vi "Write (recursive).vi"(7 "LoopData in":T3, 9 "Options":T1, 10 "Anything":variant, 11 "TagPath":string[](array[string])) -> (0 "error out":errorcluster, 3 "Tree Items":T4[](array[typedef]), 5 "LoopData out":T3)   [LabVIEW 2020, in "BlueVariantView.lvlib"]
uses:
  BlueVariantView.lvlib
  API/Typedefs/TreeData.ctl
  LoopData.ctl
  API/Typedefs/Options.ctl
  IsErrorCluster.vi
  SymbolEnumToIndex.vi
  StringArrayToScalar.vi
  <vilib>/Utility/Data Type/Get Cluster Information.vi
  <userlib>/_OpenG.lib/lvdata/lvdata.llb/Array Size(s)__ogtk.vi
  <vilib>/Utility/error.llb/Trim Whitespace.vi
  <vilib>/Utility/error.llb/Error Cluster From Error Code.vi
  <vilib>/Utility/LVClass/Get LV Class Name.vi
  <vilib>/PNR/LabVIEW Composition/Composition/Decompose LabVIEW Object.vi
  <vilib>/PNR/LabVIEW Composition/Composition/Decompose Map.vi
  <vilib>/Utility/Data Type/Get Numeric Information.vi
  <userlib>/_OpenG.lib/lvdata/lvdata.llb/Get Physical Units__ogtk.vi
  <vilib>/ErrorRing/Error Ring.xnode
  <vilib>/Utility/Data Type/NI_Data Type.lvlib
  <vilib>/PNR/LabVIEW Composition/Composition/Composition.lvlib
  API/Typedefs/ValueOptions.ctl
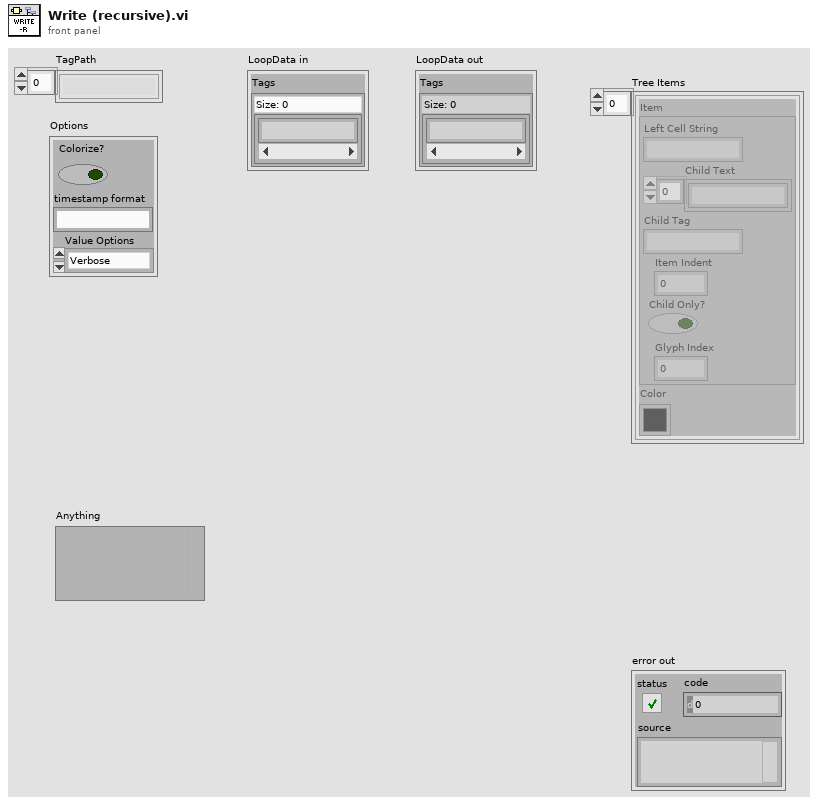
[diagram p1: front panel]
types:
  T1 = typedef "BlueVariantView.lvlib/Options.ctl" = cluster{"Colorize?":bool, "timestamp format":string, "Value Options":T2}
  T2 = typedef "BlueVariantView.lvlib/ValueOptions.ctl" = enum16{"Verbose", "Data only"}
  T3 = typedef "BlueVariantView.lvlib/LoopData.ctl" = cluster{"Tags":set{string}}
  T4 = typedef "BlueVariantView.lvlib/TreeData.ctl" = cluster{"Item":cluster{"Left Cell String":string, "Child Text":string[], "Child Tag":string, "Item Indent":i32, "Child Only?":bool, "Glyph Index":i32}, "Color":u32}
  T5 = typedef "NI_Data Type.lvlib/Data Type.ctl" = enum8{"Invalid Type", "Void", "I8", "I16", "I32", "I64", "U8", "U16", "U32", "U64", "Single Float", "Double Float", "Extended Float", "Single Complex", "Double Complex", "Extended Complex", "Enum U8", "Enum U16", "Enum U32", "Enum U64", "Single Float With Unit", "Double Float With Unit", "Extended Float With Unit", "Single Complex with Unit", "Double Complex with Unit", "Extended Complex with Unit", "Boolean", "String", "Path", "Picture", "Tag", "Array", "Cluster", "Variant", "LV Variant", "Waveform", "Timestamp", "Digital Waveform", "Digital Data", "ExpressData", "Refnum", "External Data", "VI", "Poly VI", "LabVIEW Class Instance", "Fixed Point", "Set Collection", "Map Collection"}
  T6 = typedef "BlueVariantView.lvlib/DecomposedObject.ctl" = cluster{"class name":string, "class version":string, "Private Data":variant}
  T7 = typedef "BlueVariantView.lvlib/DecomposedMap.ctl" = cluster{"Key":variant, "Value":variant}
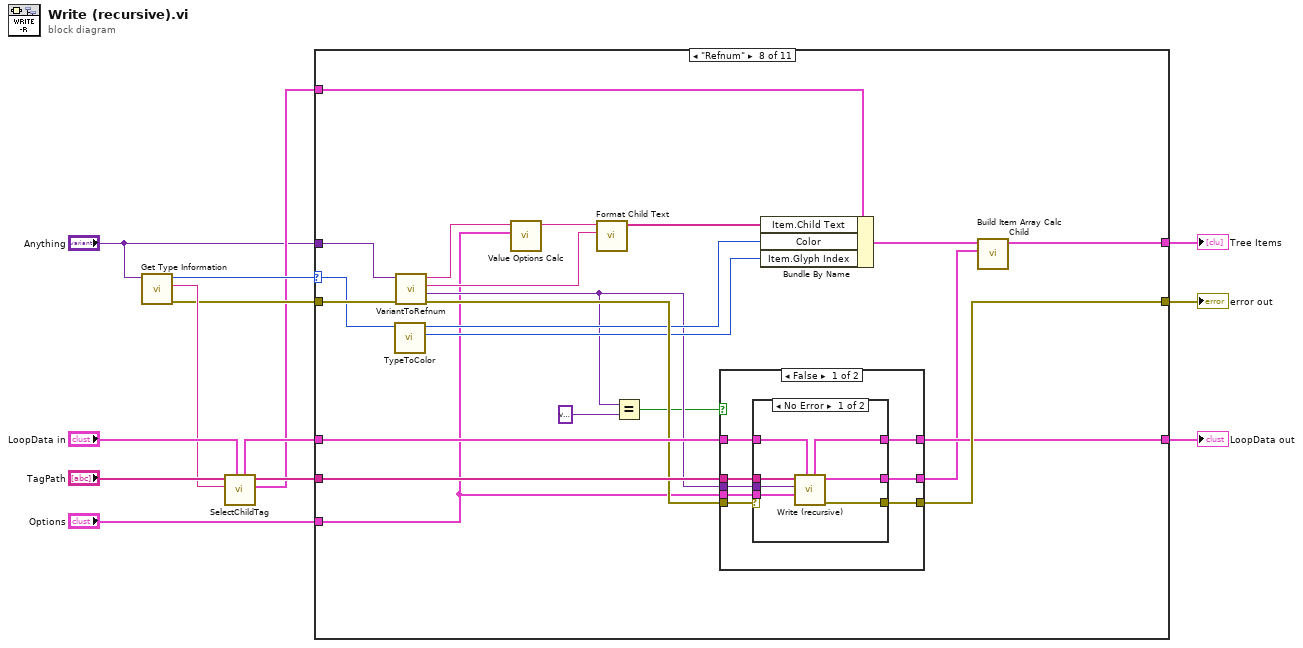
[diagram p0: block diagram]
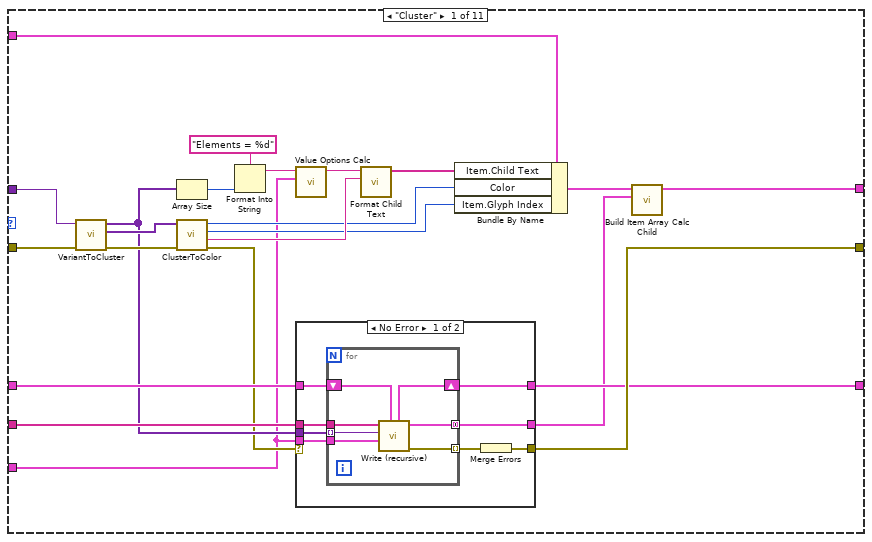
[diagram p2: hidden frame]
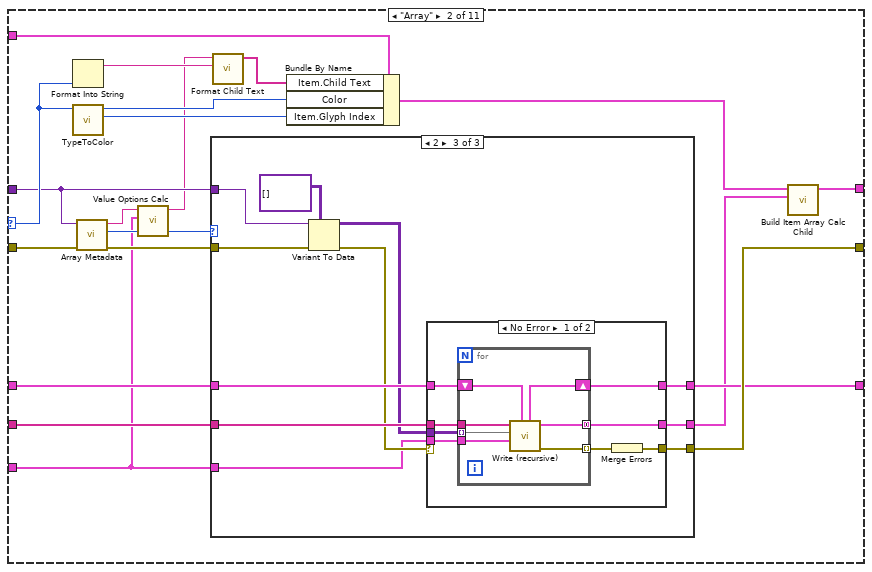
[diagram p4: hidden frame]
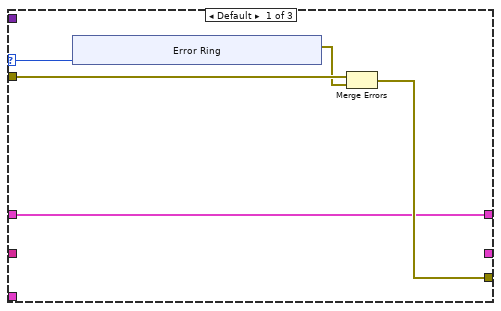
[diagram p5: hidden frame]
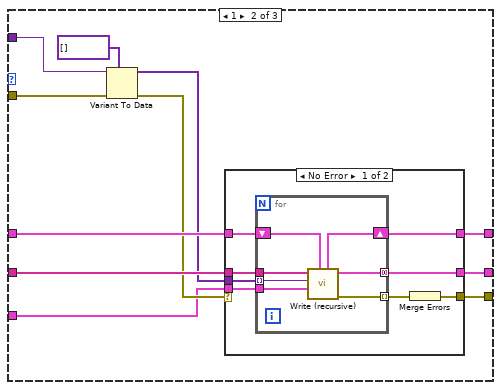
[diagram p6: hidden frame]
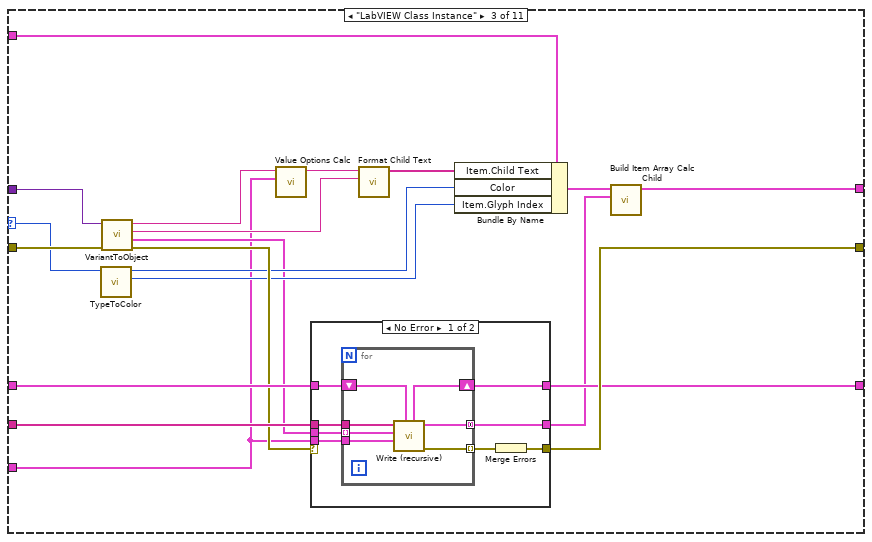
[diagram p9: hidden frame]
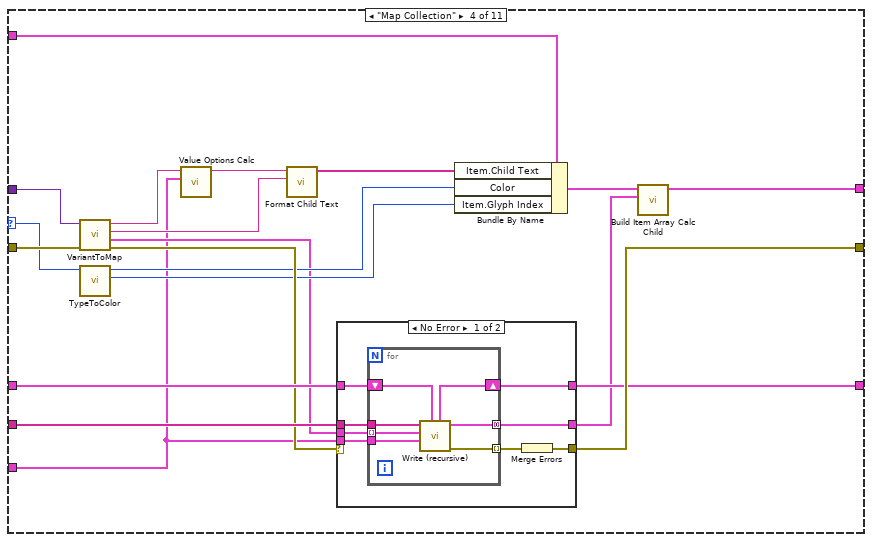
[diagram p11: hidden frame]
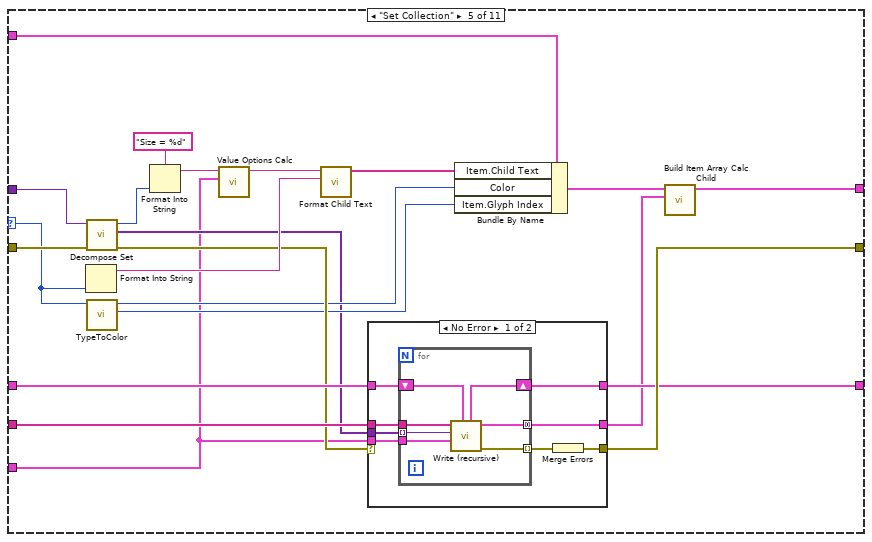
[diagram p13: hidden frame]
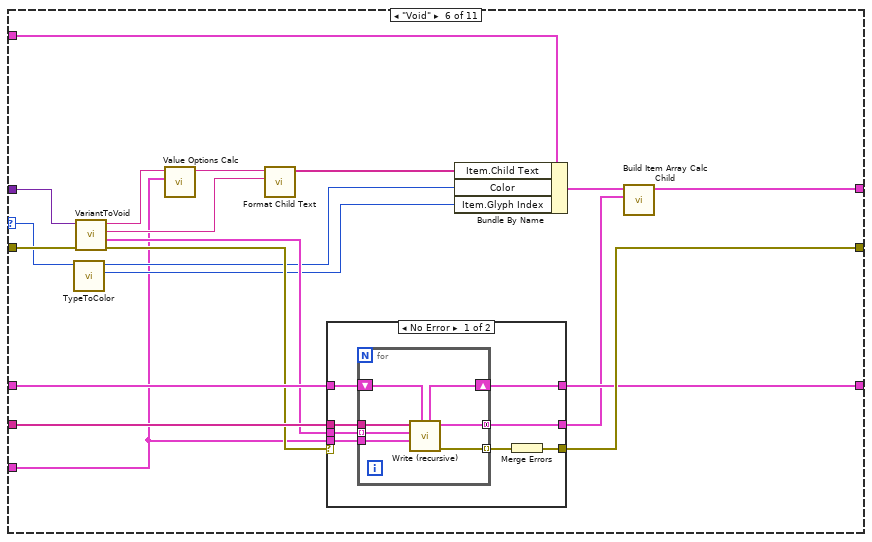
[diagram p15: hidden frame]
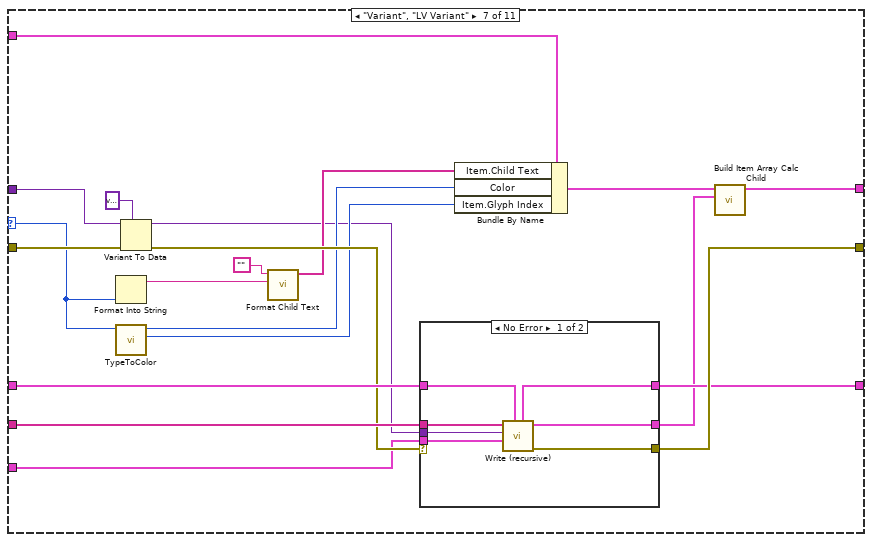
[diagram p17: hidden frame]
diagram:
  n1 = call <vilib>:"Get Type Information.vi"("variant"="Anything") -> ("error out"=w9:errorcluster, "name"=w11:string, "type"=w10:T5)  [unwired: 6 in, 2 out]
  n2 = call "SelectChildTag.vi"("LoopData in"="LoopData in", "Name"=w11, "TagPath in"="TagPath") -> ("Item"=w6:T4, "TagPath out"=w8:string[], "LoopData out"=w7:T3)  [unwired: 6 in]
  n3 = case shown="\"Refnum\"" w10 {
    selector: w10 -> [_ w67 w154 w188 w227 w263 w301 w332 w368 w381 w396]
    tunnel: w9 -> [w36 w68 w156 w193 w229 w269 w305 w337 w371 w383 w399]
    tunnel: w8 -> [w33 w72 w160 w197 w236 w273 w310 w341 _ _ _]
    tunnel: w7 -> [w32 w71 w159 w196 w235 w272 w309 w340 w365 w388 w404]
    tunnel: w6 -> [w23 w69 w157 w194 w233 w270 w307 w338 w374 w392 w408]
    tunnel: "Anything" -> [w35 w65 w155 w192 w228 w268 w306 w336 w370 w385 w398]
    tunnel: [w34 w73 w161 w198 w237 w274 w311 w342 w364 w382 w400] -> w4
    tunnel: [w31 w70 w158 w195 w234 w271 w308 w339 w365 w388 w404] -> w3
    tunnel: [w17 w59 w145 w182 w219 w258 w293 w324 w362 w386 w402] -> w2
    tunnel: "Options" -> [w14 w54 w142 w180 w216 w255 w292 w321 _ w377 _]
    frame "Cluster" {
      n4 = call "VariantToCluster.vi"("error in (no error)"=w36, "Cluster"=w35) -> ("error out"=w26:errorcluster, "cluster elements info"=w25:variant[], "Cluster elements"=w21:variant[])  [unwired: 7 in]
      n5 = Array Size(array=w21) -> (size(s)=w24:i32)
      n6 = call "ClusterToColor.vi"("error in (no error)"=w26, "cluster elements info"=w25) -> ("error out"=w20:errorcluster, "Type"=w29:string, "ItemSyms"=w22:i32, "Color"=w27:u32)  [unwired: 6 in]
      n7 = Format Into String(format string="Elements = %d", w24) -> (resulting string=w16:string)  [unwired: 2 in, 1 out]
      n8 = call "Value Options Calc.vi"("Options"=w14, "Value"=w16) -> ("Value"=w15:string)  [unwired: 9 in]
      n9 = case shown="No Error" w20 {
        selector: w20 -> [_ w53]
        tunnel: [w43 w53] -> w34
        tunnel: w21 -> [w42 _]
        tunnel: w33 -> [w41 _]
        tunnel: w32 -> [w40 w52]
        tunnel: [w39 _] -> w18
        tunnel: [w38 w52] -> w31
        tunnel: w14 -> [w37 _]
        frame No Error {
          n10 = for {
            tunnel: [w51] -> w44 mode=indexing
            tunnel: w42 -> [w50] mode=indexing
            tunnel: w41 -> [w49]
            shift-right: [w47] -> w38
            shift-left: w40 -> [w48]
            tunnel: [w46] -> w39 mode=concatenating
            tunnel: w37 -> [w45]
            n11 = call "Write (recursive).vi"("LoopData in"=w48, "Options"=w45, "Anything"=w50, "TagPath"=w49) -> ("error out"=w51:errorcluster, "Tree Items"=w46:T4[], "LoopData out"=w47:T3)  [unwired: 5 in]
          }
          n12 = Merge Errors(w44) -> (w43:errorcluster)
        }
        frame Error {
        }
      }
      n13 = call "Format Child Text.vi"("Type"=w29, "Value"=w15) -> ("Child Text"=w28:string[])  [unwired: 9 in]
      n14 = Bundle By Name(cluster=w23, "Item.Child Text"=w28, "Color"=w27, "Item.Glyph Index"=w22) -> (w19:T4)
      n15 = call "Build Item Array Calc Child.vi"("Children items"=w18, "Parent Item"=w19) -> ("Concatenated items"=w17:T4[])  [unwired: 9 in]
    }
    frame "Array" {
      n16 = Format Into String(w67) -> (resulting string=w63:string)  [unwired: 3 in, 1 out]
      n17 = call "TypeToColor.vi"("type"=w67) -> ("ItemSyms"=w61:i32, "Color"=w62:u32)  [unwired: 9 in]
      n18 = call "Array Metadata.vi"("error in (no error)"=w68, "Array"=w65) -> ("error out"=w66:errorcluster, "number of dimensions"=w60:u32, "Value"=w56:string)  [unwired: 7 in]
      n19 = call "Value Options Calc.vi"("Options"=w54, "Value"=w56) -> ("Value"=w55:string)  [unwired: 9 in]
      n20 = case shown="2" w60 {
        selector: w60 -> [w78 _ _]
        tunnel: [w75 w96 w124] -> w73
        tunnel: w72 -> [_ w95 w123]
        tunnel: w71 -> [w74 w94 w122]
        tunnel: [w74 w93 w121] -> w70
        tunnel: [_ w92 w120] -> w58
        tunnel: w66 -> [w77 w90 w118]
        tunnel: w65 -> [_ w89 w117]
        tunnel: w54 -> [_ w86 w114]
        frame Default {
          n21 = xnode "Error Ring"("parameter 0"=w78) -> ("error out"=w76:errorcluster)
          n22 = Merge Errors(w77, w76) -> (w75:errorcluster)
        }
        frame 1 {
          n23 = Variant To Data(error in=w90, type=variant[] [], Variant=w89) -> (data=w88:variant[], error out=w87:errorcluster)
          n24 = case shown="No Error" w87 {
            selector: w87 -> [_ w113]
            tunnel: [w103 w113] -> w96
            tunnel: w88 -> [w102 _]
            tunnel: w95 -> [w101 _]
            tunnel: w94 -> [w100 w112]
            tunnel: [w99 _] -> w92
            tunnel: [w98 w112] -> w93
            tunnel: w86 -> [w97 _]
            frame No Error {
              n25 = for {
                tunnel: [w111] -> w104 mode=indexing
                tunnel: w102 -> [w110] mode=indexing
                tunnel: w101 -> [w109]
                shift-right: [w107] -> w98
                shift-left: w100 -> [w108]
                tunnel: [w106] -> w99 mode=concatenating
                tunnel: w97 -> [w105]
                n26 = call "Write (recursive).vi"("LoopData in"=w108, "Options"=w105, "Anything"=w110, "TagPath"=w109) -> ("error out"=w111:errorcluster, "Tree Items"=w106:T4[], "LoopData out"=w107:T3)  [unwired: 5 in]
              }
              n27 = Merge Errors(w104) -> (w103:errorcluster)
            }
            frame Error {
            }
          }
        }
        frame 2 {
          n28 = Variant To Data(error in=w118, type=variant[][] [], Variant=w117) -> (data=w116:variant[][], error out=w115:errorcluster)
          n29 = case shown="No Error" w115 {
            selector: w115 -> [_ w141]
            tunnel: [w131 w141] -> w124
            tunnel: w116 -> [w130 _]
            tunnel: w123 -> [w129 _]
            tunnel: w122 -> [w128 w140]
            tunnel: [w127 _] -> w120
            tunnel: [w126 w140] -> w121
            tunnel: w114 -> [w125 _]
            frame No Error {
              n30 = for {
                tunnel: [w139] -> w132 mode=indexing
                tunnel: w130 -> [w138] mode=indexing
                tunnel: w129 -> [w137]
                shift-right: [w135] -> w126
                shift-left: w128 -> [w136]
                tunnel: [w134] -> w127 mode=concatenating
                tunnel: w125 -> [w133]
                n31 = call "Write (recursive).vi"("LoopData in"=w136, "Options"=w133, "Anything"=w138, "TagPath"=w137) -> ("error out"=w139:errorcluster, "Tree Items"=w134:T4[], "LoopData out"=w135:T3)  [unwired: 5 in]
              }
              n32 = Merge Errors(w132) -> (w131:errorcluster)
            }
            frame Error {
            }
          }
        }
      }
      n33 = call "Format Child Text.vi"("Type"=w63, "Value"=w55) -> ("Child Text"=w64:string[])  [unwired: 9 in]
      n34 = Bundle By Name(cluster=w69, "Item.Child Text"=w64, "Color"=w62, "Item.Glyph Index"=w61) -> (w57:T4)
      n35 = call "Build Item Array Calc Child.vi"("Children items"=w58, "Parent Item"=w57) -> ("Concatenated items"=w59:T4[])  [unwired: 9 in]
    }
    frame "LabVIEW Class Instance" {
      n36 = call "TypeToColor.vi"("type"=w154) -> ("ItemSyms"=w149:i32, "Color"=w150:u32)  [unwired: 9 in]
      n37 = call "VariantToObject.vi"("error in (no error)"=w156, "Object"=w155) -> ("error out"=w151:errorcluster, "DecomposedObject"=w148:T6[], "Type"=w152:string, "Value"=w144:string)  [unwired: 6 in]
      n38 = call "Value Options Calc.vi"("Options"=w142, "Value"=w144) -> ("Value"=w143:string)  [unwired: 9 in]
      n39 = case shown="No Error" w151 {
        selector: w151 -> [_ w178]
        tunnel: [w168 w178] -> w161
        tunnel: w148 -> [w167 _]
        tunnel: w160 -> [w166 _]
        tunnel: w159 -> [w165 w177]
        tunnel: [w164 _] -> w146
        tunnel: [w163 w177] -> w158
        tunnel: w142 -> [w162 _]
        frame No Error {
          n40 = for {
            tunnel: [w176] -> w169 mode=indexing
            tunnel: w167 -> [w175] mode=indexing
            tunnel: w166 -> [w174]
            shift-right: [w172] -> w163
            shift-left: w165 -> [w173]
            tunnel: [w171] -> w164 mode=concatenating
            tunnel: w162 -> [w170]
            n41 = call "Write (recursive).vi"("LoopData in"=w173, "Options"=w170, "Anything"=w175, "TagPath"=w174) -> ("error out"=w176:errorcluster, "Tree Items"=w171:T4[], "LoopData out"=w172:T3)  [unwired: 5 in]
          }
          n42 = Merge Errors(w169) -> (w168:errorcluster)
        }
        frame Error {
        }
      }
      n43 = call "Format Child Text.vi"("Type"=w152, "Value"=w143) -> ("Child Text"=w153:string[])  [unwired: 9 in]
      n44 = Bundle By Name(cluster=w157, "Item.Child Text"=w153, "Color"=w150, "Item.Glyph Index"=w149) -> (w147:T4)
      n45 = call "Build Item Array Calc Child.vi"("Children items"=w146, "Parent Item"=w147) -> ("Concatenated items"=w145:T4[])  [unwired: 9 in]
    }
    frame "Map Collection" {
      n46 = call "VariantToMap.vi"("error in (no error)"=w193, "Map"=w192) -> ("error out"=w189:errorcluster, "DecomposedMap"=w185:T7[], "Type"=w190:string, "Value"=w181:string)  [unwired: 6 in]
      n47 = call "TypeToColor.vi"("type"=w188) -> ("ItemSyms"=w186:i32, "Color"=w187:u32)  [unwired: 9 in]
      n48 = call "Value Options Calc.vi"("Options"=w180, "Value"=w181) -> ("Value"=w179:string)  [unwired: 9 in]
      n49 = call "Format Child Text.vi"("Type"=w190, "Value"=w179) -> ("Child Text"=w191:string[])  [unwired: 9 in]
      n50 = case shown="No Error" w189 {
        selector: w189 -> [_ w215]
        tunnel: [w205 w215] -> w198
        tunnel: w185 -> [w204 _]
        tunnel: w197 -> [w203 _]
        tunnel: w196 -> [w202 w214]
        tunnel: [w201 _] -> w184
        tunnel: [w200 w214] -> w195
        tunnel: w180 -> [w199 _]
        frame No Error {
          n51 = for {
            tunnel: [w213] -> w206 mode=indexing
            tunnel: w204 -> [w212] mode=indexing
            tunnel: w203 -> [w211]
            shift-right: [w209] -> w200
            shift-left: w202 -> [w210]
            tunnel: [w208] -> w201 mode=concatenating
            tunnel: w199 -> [w207]
            n52 = call "Write (recursive).vi"("LoopData in"=w210, "Options"=w207, "Anything"=w212, "TagPath"=w211) -> ("error out"=w213:errorcluster, "Tree Items"=w208:T4[], "LoopData out"=w209:T3)  [unwired: 5 in]
          }
          n53 = Merge Errors(w206) -> (w205:errorcluster)
        }
        frame Error {
        }
      }
      n54 = Bundle By Name(cluster=w194, "Item.Child Text"=w191, "Color"=w187, "Item.Glyph Index"=w186) -> (w183:T4)
      n55 = call "Build Item Array Calc Child.vi"("Children items"=w184, "Parent Item"=w183) -> ("Concatenated items"=w182:T4[])  [unwired: 9 in]
    }
    frame "Set Collection" {
      n56 = Format Into String(w227) -> (resulting string=w231:string)  [unwired: 3 in, 1 out]
      n57 = call <vilib>:"Decompose Set.vi"("error in (no error)"=w229, "Variant"=w228) -> ("error out"=w226:errorcluster, "Elements"=w222:variant[], "Size"=w230:i32)  [unwired: 7 in]
      n58 = call "TypeToColor.vi"("type"=w227) -> ("ItemSyms"=w223:i32, "Color"=w224:u32)  [unwired: 9 in]
      n59 = Format Into String(format string="Size = %d", w230) -> (resulting string=w218:string)  [unwired: 2 in, 1 out]
      n60 = call "Value Options Calc.vi"("Options"=w216, "Value"=w218) -> ("Value"=w217:string)  [unwired: 9 in]
      n61 = call "Format Child Text.vi"("Type"=w231, "Value"=w217) -> ("Child Text"=w225:string[])  [unwired: 9 in]
      n62 = case shown="No Error" w226 {
        selector: w226 -> [_ w254]
        tunnel: [w244 w254] -> w237
        tunnel: w222 -> [w243 _]
        tunnel: w236 -> [w242 _]
        tunnel: w235 -> [w241 w253]
        tunnel: [w240 _] -> w221
        tunnel: [w239 w253] -> w234
        tunnel: w216 -> [w238 _]
        frame No Error {
          n63 = for {
            tunnel: [w252] -> w245 mode=indexing
            tunnel: w243 -> [w251] mode=indexing
            tunnel: w242 -> [w250]
            shift-right: [w248] -> w239
            shift-left: w241 -> [w249]
            tunnel: [w247] -> w240 mode=concatenating
            tunnel: w238 -> [w246]
            n64 = call "Write (recursive).vi"("LoopData in"=w249, "Options"=w246, "Anything"=w251, "TagPath"=w250) -> ("error out"=w252:errorcluster, "Tree Items"=w247:T4[], "LoopData out"=w248:T3)  [unwired: 5 in]
          }
          n65 = Merge Errors(w245) -> (w244:errorcluster)
        }
        frame Error {
        }
      }
      n66 = Bundle By Name(cluster=w233, "Item.Child Text"=w225, "Color"=w224, "Item.Glyph Index"=w223) -> (w220:T4)
      n67 = call "Build Item Array Calc Child.vi"("Children items"=w221, "Parent Item"=w220) -> ("Concatenated items"=w219:T4[])  [unwired: 9 in]
    }
    frame "Void" {
      n68 = call "TypeToColor.vi"("type"=w263) -> ("ItemSyms"=w261:i32, "Color"=w262:u32)  [unwired: 9 in]
      n69 = call "VariantToVoid.vi"("error in (no error)"=w269, "Void"=w268) -> ("error out"=w265:errorcluster, "DecomposedVariant"=w264:T7[], "Type"=w266:string, "Value"=w257:string)  [unwired: 6 in]
      n70 = call "Value Options Calc.vi"("Options"=w255, "Value"=w257) -> ("Value"=w256:string)  [unwired: 9 in]
      n71 = call "Format Child Text.vi"("Type"=w266, "Value"=w256) -> ("Child Text"=w267:string[])  [unwired: 9 in]
      n72 = case shown="No Error" w265 {
        selector: w265 -> [_ w291]
        tunnel: [w281 w291] -> w274
        tunnel: w264 -> [w280 _]
        tunnel: w273 -> [w279 _]
        tunnel: w272 -> [w278 w290]
        tunnel: [w277 _] -> w260
        tunnel: [w276 w290] -> w271
        tunnel: w255 -> [w275 _]
        frame No Error {
          n73 = for {
            tunnel: [w289] -> w282 mode=indexing
            tunnel: w280 -> [w288] mode=indexing
            tunnel: w279 -> [w287]
            shift-right: [w285] -> w276
            shift-left: w278 -> [w286]
            tunnel: [w284] -> w277 mode=concatenating
            tunnel: w275 -> [w283]
            n74 = call "Write (recursive).vi"("LoopData in"=w286, "Options"=w283, "Anything"=w288, "TagPath"=w287) -> ("error out"=w289:errorcluster, "Tree Items"=w284:T4[], "LoopData out"=w285:T3)  [unwired: 5 in]
          }
          n75 = Merge Errors(w282) -> (w281:errorcluster)
        }
        frame Error {
        }
      }
      n76 = Bundle By Name(cluster=w270, "Item.Child Text"=w267, "Color"=w262, "Item.Glyph Index"=w261) -> (w259:T4)
      n77 = call "Build Item Array Calc Child.vi"("Children items"=w260, "Parent Item"=w259) -> ("Concatenated items"=w258:T4[])  [unwired: 9 in]
    }
    frame "Variant", "LV Variant" {
      n78 = Format Into String(w301) -> (resulting string=w303:string)  [unwired: 3 in, 1 out]
      n79 = call "TypeToColor.vi"("type"=w301) -> ("ItemSyms"=w298:i32, "Color"=w299:u32)  [unwired: 9 in]
      n80 = Variant To Data(error in=w305, type=variant ("Anything"), Variant=w306) -> (data=w297:variant, error out=w304:errorcluster)
      n81 = call "Format Child Text.vi"("Type"=w303, "Value"="") -> ("Child Text"=w300:string[])  [unwired: 9 in]
      n82 = case shown="No Error" w304 {
        selector: w304 -> [_ w320]
        tunnel: [w313 w320] -> w311
        tunnel: w297 -> [w318 _]
        tunnel: w310 -> [w317 _]
        tunnel: w309 -> [w316 w319]
        tunnel: [w315 _] -> w295
        tunnel: [w314 w319] -> w308
        tunnel: w292 -> [w312 _]
        frame No Error {
          n83 = call "Write (recursive).vi"("LoopData in"=w316, "Options"=w312, "Anything"=w318, "TagPath"=w317) -> ("error out"=w313:errorcluster, "Tree Items"=w315:T4[], "LoopData out"=w314:T3)  [unwired: 5 in]
        }
        frame Error {
        }
      }
      n84 = Bundle By Name(cluster=w307, "Item.Child Text"=w300, "Color"=w299, "Item.Glyph Index"=w298) -> (w294:T4)
      n85 = call "Build Item Array Calc Child.vi"("Children items"=w295, "Parent Item"=w294) -> ("Concatenated items"=w293:T4[])  [unwired: 9 in]
    }
    frame "Refnum" {
      n86 = call "TypeToColor.vi"("type"=w332) -> ("ItemSyms"=w330:i32, "Color"=w331:u32)  [unwired: 9 in]
      n87 = call "VariantToRefnum.vi"("error in (no error)"=w337, "Refnum"=w336) -> ("error out"=w333:errorcluster, "strict type"=w328:variant, "type"=w335:string, "value"=w323:string)  [unwired: 6 in]
      n88 = call "Value Options Calc.vi"("Options"=w321, "Value"=w323) -> ("Value"=w322:string)  [unwired: 9 in]
      n89 = call "Format Child Text.vi"("Type"=w335, "Value"=w322) -> ("Child Text"=w334:string[])  [unwired: 9 in]
      n90 = Equal?(x=w328, y=variant ("strict type")) -> (x = y?=w327:bool)
      n91 = case shown="False" w327 {
        tunnel: [w350 w360] -> w342
        tunnel: w341 -> [w349 _]
        tunnel: w340 -> [w348 w361]
        tunnel: [w347 w361] -> w339
        tunnel: [w346 _] -> w325
        tunnel: w333 -> [w345 w360]
        tunnel: w328 -> [w344 _]
        tunnel: w321 -> [w343 _]
        frame False {
          n92 = case shown="No Error" w345 {
            selector: w345 -> [_ w359]
            tunnel: [w352 w359] -> w350
            tunnel: w344 -> [w357 _]
            tunnel: w349 -> [w356 _]
            tunnel: w348 -> [w355 w358]
            tunnel: [w354 _] -> w346
            tunnel: [w353 w358] -> w347
            tunnel: w343 -> [w351 _]
            frame No Error {
              n93 = call "Write (recursive).vi"("LoopData in"=w355, "Options"=w351, "Anything"=w357, "TagPath"=w356) -> ("error out"=w352:errorcluster, "Tree Items"=w354:T4[], "LoopData out"=w353:T3)  [unwired: 5 in]
            }
            frame Error {
            }
          }
        }
        frame True {
        }
      }
      n94 = Bundle By Name(cluster=w338, "Item.Child Text"=w334, "Color"=w331, "Item.Glyph Index"=w330) -> (w326:T4)
      n95 = call "Build Item Array Calc Child.vi"("Children items"=w325, "Parent Item"=w326) -> ("Concatenated items"=w324:T4[])  [unwired: 9 in]
    }
    frame "I8".."Path" {
      n96 = call "ScalarVariantToData.vi"("error in (no error)"=w371, "type"=w368, "Variant"=w370) -> ("error out"=w364:errorcluster, "Type"=w372:string, "Value"=w373:string)  [unwired: 6 in]
      n97 = call "TypeToColor.vi"("type"=w368) -> ("ItemSyms"=w366:i32, "Color"=w367:u32)  [unwired: 9 in]
      n98 = call "Format Child Text.vi"("Type"=w372, "Value"=w373) -> ("Child Text"=w369:string[])  [unwired: 9 in]
      n99 = Bundle By Name(cluster=w374, "Item.Child Text"=w369, "Color"=w367, "Item.Glyph Index"=w366) -> (w363:T4)
      n100 = call "Build Item Array Calc Child.vi"("Parent Item"=w363) -> ("Concatenated items"=w362:T4[])  [unwired: 10 in]
    }
    frame "Timestamp" {
      n101 = Unbundle By Name(w377) -> ("timestamp format"=w376:string)
      n102 = Variant To Data(error in=w383, type=timestamp(0 s since 1904-01-01), Variant=w385) -> (data=w379:timestamp, error out=w382:errorcluster)
      n103 = Format Into String(w381) -> (resulting string=w380:string)  [unwired: 3 in, 1 out]
      n104 = call "TypeToColor.vi"("type"=w381) -> ("ItemSyms"=w389:i32, "Color"=w390:u32)  [unwired: 9 in]
      n105 = case shown="\"\"" w376 {
        selector: w376 -> [w393 _]
        tunnel: [w393 "%H:%M:%S%.3u %d/%m/%Y" ("time format string (%c)")] -> w375
        frame Default {
        }
        frame "" {
        }
      }
      n106 = Format Date/Time String(time format string (%c)=w375, seconds (now)=w379) -> (date/time string=w378:string)  [unwired: 1 in]
      n107 = call "Format Child Text.vi"("Type"=w380, "Value"=w378) -> ("Child Text"=w391:string[])  [unwired: 9 in]
      n108 = Bundle By Name(cluster=w392, "Item.Child Text"=w391, "Color"=w390, "Item.Glyph Index"=w389) -> (w387:T4)
      n109 = call "Build Item Array Calc Child.vi"("Parent Item"=w387) -> ("Concatenated items"=w386:T4[])  [unwired: 10 in]
    }
    frame Default {
      n110 = Format Into String(w396) -> (resulting string=w395:string)  [unwired: 3 in, 1 out]
      n111 = call "TypeToColor.vi"("type"=w396) -> ("ItemSyms"=w405:i32, "Color"=w406:u32)  [unwired: 9 in]
      n112 = Flatten To String(anything=w398, prepend array or string size? (T)=FALSE, error in (no error)=w399) -> (data string=w397:string, error out=w400:errorcluster)  [unwired: 1 in, 1 out]
      n113 = call "Format Child Text.vi"("Type"=w395, "Value"=w397) -> ("Child Text"=w407:string[])  [unwired: 9 in]
      n114 = Bundle By Name(cluster=w408, "Item.Child Text"=w407, "Color"=w406, "Item.Glyph Index"=w405) -> (w403:T4)
      n115 = call "Build Item Array Calc Child.vi"("Parent Item"=w403) -> ("Concatenated items"=w402:T4[])  [unwired: 10 in]
    }
  }
  "error out" <- w4
  "Tree Items" <- w2
  "LoopData out" <- w3
